vi "RemoteVI Close Submenus.vi"(0 "hWnd":u64, 5 "count":i32, 11 "error in":errorcluster) -> (15 "error out":errorcluster)   [LabVIEW 2020, in "RemoteVI.lvlib"]
doc: "Closes the count deepest submenus of an open LabVIEW menu chain, as moving the pointer back to a parent menu does locally: posts one VK_LEFT (scan code 0x4B, extended) per submenu to the panel window with RemoteVI Post Menu Key.vi, each waiting until LabVIEW has handled it. VK_LEFT closes the deepest open submenu and leaves its parent's highlight on the item that opened it (measured). A custom popup such as the colour picker takes no keys and is not closed by this. No VI Server call."
uses:
  RemoteVI.lvlib
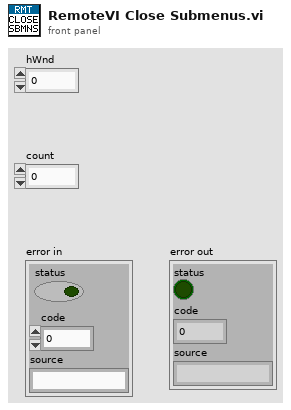
[diagram p1: front panel]
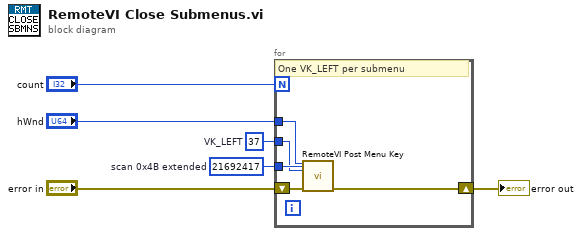
[diagram p0: block diagram]
diagram:
  w5 = i64 21692417  # scan 0x4B extended
  w4 = u64 37  # VK_LEFT
  n1 = for {
    N: "count" -> [_]
    tunnel: "hWnd" -> [w7]
    tunnel: w4 -> [w8]
    tunnel: w5 -> [w9]
    shift-right: [w11] -> w6
    shift-left: "error in" -> [w10]
    # "One VK_LEFT per submenu"
    n2 = call "RemoteVI Post Menu Key.vi"("hWnd"=w7, "vk"=w8, "key lParam"=w9, "error in"=w10) -> ("error out"=w11:errorcluster)  [unwired: 11 in]
  }
  "error out" <- w6
